vi "Inspect_Surface.vi"(9 "Max Dark Pixels":i16, 10 "Dark Level":dbl, 11 "Image":u8[][](array[numeric])) -> (1 "Surface Defect":string, 2 "Surface OK":bool, 3 "Dark Pixels":i16)   [LabVIEW 2018]
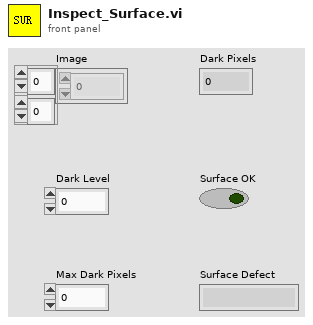
[diagram p1: front panel]
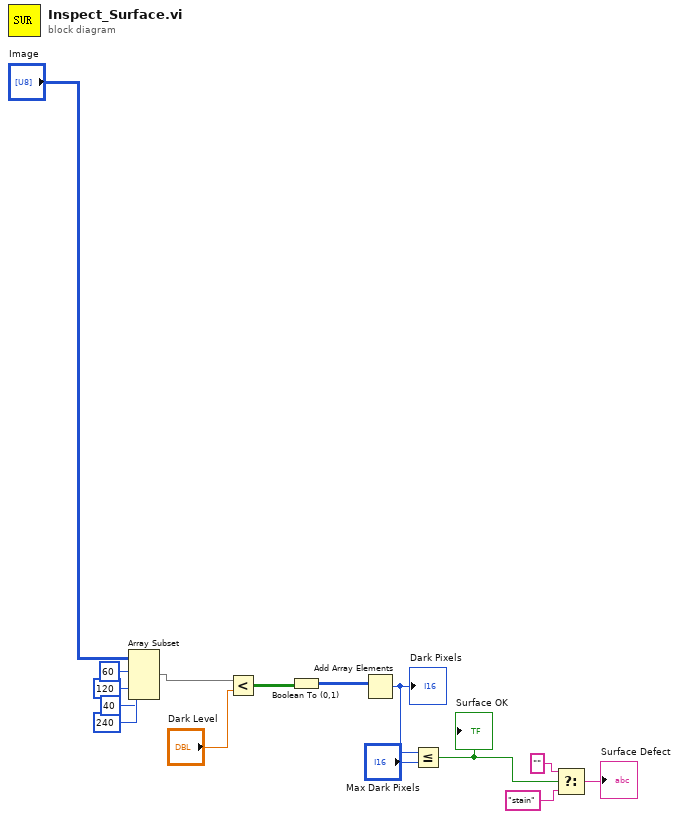
[diagram p0: block diagram]
diagram:
  n1 = Array Subset(array="Image", index (row)=60 ("index"), length (row)=120 ("length"), index (col)=40 ("index"), length (col)=240 ("length")) -> (w6:u8[][])
  n2 = Less?(x=w6, y="Dark Level") -> (x < y?=w7:bool[][])
  n3 = Boolean To (0,1)(Boolean=w7) -> (0, 1=w8:i16[][])
  n4 = Add Array Elements(numeric array=w8) -> (sum=w9:i16)
  "Dark Pixels" <- w9
  n5 = Less Or Equal?(x=w9, y="Max Dark Pixels") -> (x <= y?=w11:bool)
  "Surface OK" <- w11
  n6 = Select(t="", s=w11, f="stain") -> (s? t:f=→"Surface Defect":string)
